vi "VIH - CHM Project - Compile HHP.vi"(7 "CHM File Path":path, 8 "error in":errorcluster, 9 "wait until completion? (T)":bool=TRUE, 10 "run minimized? (T)":bool=TRUE, 11 "HHP File Path":path) -> (0 "error out":errorcluster, 1 "return code":i32, 2 "Log":string)   [LabVIEW 2014]
doc: "::: VI Helpeks :::\nCopyright (c) 2000-2026 Konstantin Shifershteyn. All rights reserved."
panel:
  # "VI Helpeks\nCopyright (c) 2012-2026 Konstantin Shifershteyn"
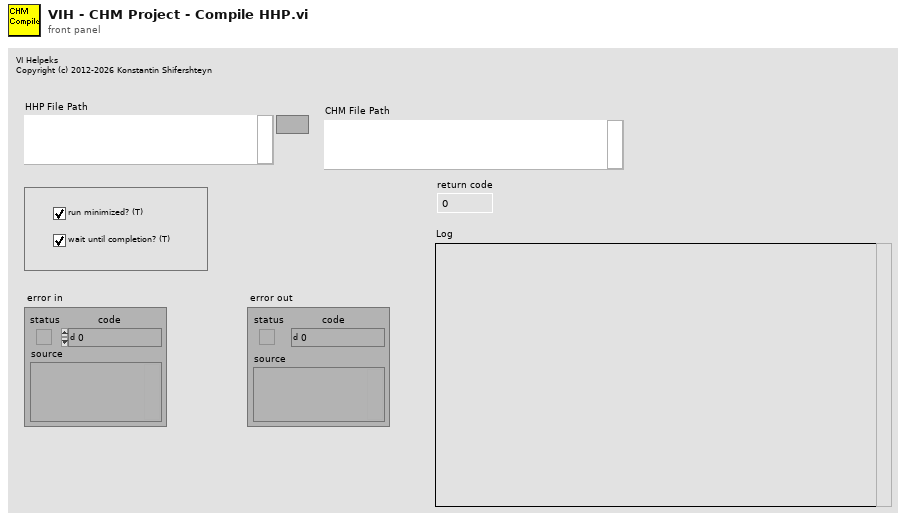
[diagram p1: front panel]
types:
  T1 = cluster{"Windows platform":bool, "HHP is associated":bool, "HHC is installed":bool}
  T2 = cluster{"Product Name":string, "Short Name":string, "Product Version":string, "Release Timestamp":string, "Developer":string, "Copyright":string}
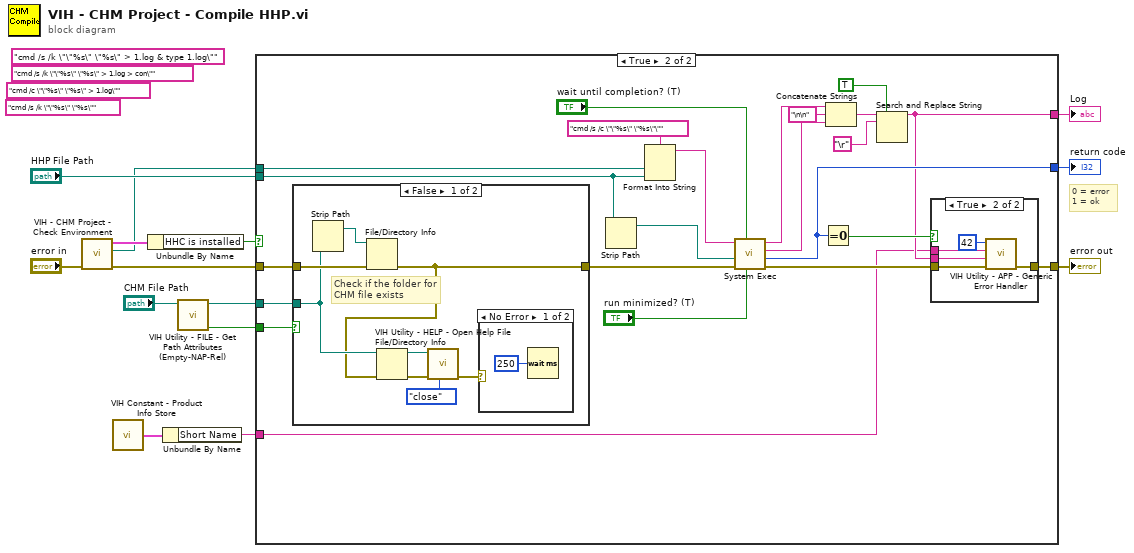
[diagram p0: block diagram]
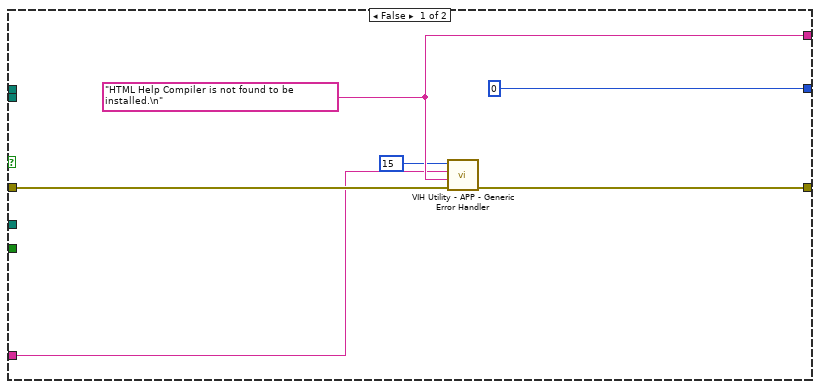
[diagram p2: hidden frame]
diagram:
  (unwired) "cmd /s /k \"\"%s\" \"%s\"" ("format string")
  (unwired) "cmd /s /k \"\"%s\" \"%s\" > 1.log & type 1.log\"" ("format string")
  (unwired) "cmd /s /k \"\"%s\" \"%s\" > 1.log > con\"" ("format string")
  (unwired) "cmd /c \"\"%s\" \"%s\" > 1.log\"" ("format string")
  # "0 = error\n1 = ok"
  n1 = call "VIH - CHM Project - Check Environment.vi"("error in"="error in") -> ("error out"=w10:errorcluster, "HHC path"=w7:path, "Flags"=w9:T1)  [unwired: 7 in, 1 out]
  n2 = call "VIH Constant - Product Info Store.vi"() -> ("Product Info"=w5:T2)
  n3 = Unbundle By Name(w9) -> ("HHC is installed"=w8:bool)
  n4 = Unbundle By Name(w5) -> ("Short Name"=w4:string)
  n5 = call "VIH Utility - FILE - Get Path Attributes (Empty-NAP-Rel).vi"("Path"="CHM File Path") -> ("Not A Path or Empty path"=w2:bool, "dup Path"=w1:path)  [unwired: 6 in, 3 out]
  n6 = case shown="True" w8 {
    tunnel: "HHP File Path" -> [_ w39]
    tunnel: [w19 w29] -> w13
    tunnel: [w18 w26] -> w12
    tunnel: w10 -> [w20 w23]
    tunnel: w7 -> [_ w31]
    tunnel: [0 ("return code") w27] -> w6
    tunnel: w4 -> [w15 w25]
    tunnel: w2 -> [_ w24]
    tunnel: w1 -> [_ w21]
    frame False {
      w18 = "HTML Help Compiler is not found to be installed.\n" ("result string")
      n7 = call "VIH Utility - APP - Generic Error Handler.vi"("error in"=w20, "error reason"=w18, "error location"=w15, "error code"=15) -> ("error out"=w19:errorcluster)  [unwired: 6 in, 1 out]
    }
    frame True {
      n8 = case shown="False" w24 {
        tunnel: w23 -> [w51 w53]
        tunnel: [w45 w53] -> w22
        tunnel: w21 -> [w49 _]
        frame False {
          # "Check if the folder for\nCHM file exists"
          n9 = Strip Path(path=w49) -> (stripped path=w50:path)  [unwired: 1 out]
          n10 = File/Directory Info(path=w50, error in=w51) -> (error out=w45:errorcluster)  [unwired: 6 out]
          n11 = File/Directory Info(path=w49, error in=w45) -> (path out=w48:path, error out=w47:errorcluster)  [unwired: 5 out]
          n12 = call "VIH Utility - HELP - Open Help File.vi"("cmd (open)"=enum16{"open", "close"}."close", "error in"=w47, "Help Path"=w48) -> ("error out"=w44:errorcluster)  [unwired: 7 in, 1 out]
          n13 = case shown="No Error" w44 {
            frame No Error {
              n14 = Wait (ms)(milliseconds to wait=u32 250) -> ()  [unwired: 1 out]
            }
            frame Error {
            }
          }
        }
        frame True {
        }
      }
      n15 = Strip Path(path=w39) -> (stripped path=w42:path)  [unwired: 1 out]
      n16 = Format Into String(format string="cmd /s /c \"\"%s\" \"%s\"\"", w31, w39) -> (resulting string=w41:string)  [unwired: 2 in, 1 out]
      n17 = call <vilib>:"System Exec.vi"("run minimized? (F)"="run minimized? (T)", "wait until completion? (T)"="wait until completion? (T)", "error in (no error)"=w22, "working directory"=w42, "command line"=w41) -> ("error out"=w30:errorcluster, "return code"=w27:i32, "standard error"=w36:string, "standard output"=w37:string)  [unwired: 3 in]
      n18 = Equal To 0?(x=w27) -> (x = 0?=w28:bool)
      n19 = Concatenate Strings(w37, "\n\n" ("string"), w36) -> (w34:string)
      n20 = Search and Replace String(replace all?=TRUE, input string=w34, search string="\r") -> (result string=w26:string)  [unwired: 5 in, 3 out]
      n21 = case shown="True" w28 {
        tunnel: w30 -> [w54 w59]
        tunnel: [w54 w58] -> w29
        tunnel: w26 -> [_ w57]
        tunnel: w25 -> [_ w55]
        frame False {
        }
        frame True {
          n22 = call "VIH Utility - APP - Generic Error Handler.vi"("error in"=w59, "error reason"=w57, "error location"=w55, "error code"=42) -> ("error out"=w58:errorcluster)  [unwired: 6 in, 1 out]
        }
      }
    }
  }
  "Log" <- w12
  "error out" <- w13
  "return code" <- w6
